vi "MenuHandler.vi"(5 "tree control":refnum<vi>, 7 "main queue":refnum<queue>, 8 "error in":errorcluster, 9 "parameters":variant, 10 "menu string":string, 11 "DMM Engine":refnum<class "DMM Engine.lvclass">) -> (0 "error out":errorcluster, 1 "refresh tree?":bool, 2 "Unhandled":bool, 3 "DMM Engine out":refnum<class "DMM Engine.lvclass">)   [LabVIEW 2025, in "DMM.lvlib" / "DMM Engine.lvclass"]
uses:
  DMM Engine.lvclass
  Users/Public/Documents/Sandia National Labs/TSS Plugin/Abstract.lvlibp/Abstract Engine/Abstract Engine.lvclass
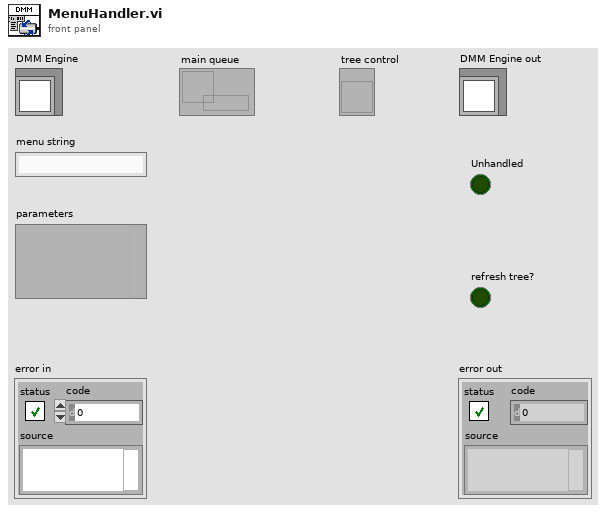
[diagram p1: front panel]
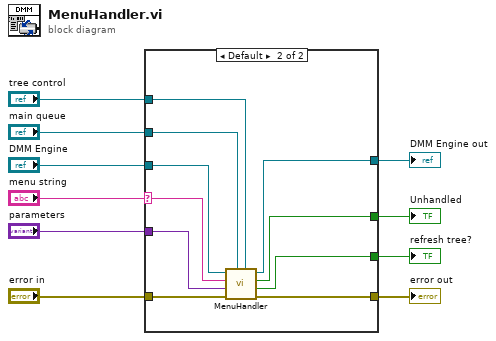
[diagram p0: block diagram]
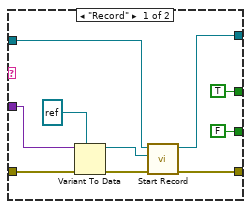
[diagram p2: hidden frame]
diagram:
  n1 = case shown="Default" "menu string" {
    selector: "menu string" -> [_ w21]
    tunnel: [w16 w30] -> w10
    tunnel: [FALSE ("refresh tree?") w29] -> w9
    tunnel: [TRUE ("Unhandled") w28] -> w8
    tunnel: [w13 w27] -> w7
    tunnel: "tree control" -> [_ w22]
    tunnel: "main queue" -> [_ w23]
    tunnel: "error in" -> [w19 w26]
    tunnel: "parameters" -> [w18 w25]
    tunnel: "DMM Engine" -> [w14 w24]
    frame "Record" {
      n2 = Variant To Data(error in=w19, type=refnum<k34> refnum ("tdms file"), Variant=w18) -> (data=w15:refnum<k34>, error out=w17:errorcluster)
      n3 = call "Start Record.vi"("error in (no error)"=w17, "tdms ref"=w15, "DMM Engine"=w14) -> ("error out"=w16:errorcluster, "DMM Engine out"=w13:refnum<class "DMM Engine.lvclass">)  [unwired: 7 in]
    }
    frame Default {
      n4 = call-parent "MenuHandler.vi"("tree control"=w22, "main queue"=w23, "error in"=w26, "parameters"=w25, "menu string"=w21, "Abstract Engine"=w24) -> ("error out"=w30:errorcluster, "refresh tree?"=w29:bool, "Unhandled"=w28:bool, "Abstract Engine out"=w27:refnum<class "DMM Engine.lvclass">)  [unwired: 2 in]
    }
  }
  "error out" <- w10
  "DMM Engine out" <- w7
  "Unhandled" <- w8
  "refresh tree?" <- w9
